vi "base color selection_N2.vi"(8 "error in":errorcluster, 11 "Sample Sequence":string="GATGATGATGATGATGAT") -> (0 "error out":errorcluster, 2 "element":string, 3 "Base All Composition":T1(array[cluster]))   [LabVIEW 2018]
panel:
  out "R STD Level array":dbl[](array[numeric])
  out "Base Species IDX array":dbl[](array[numeric])
  out "Base name array":string[](array[string])
  out "Base Color array":u32[](array[numeric])
  out "R Base Level array":dbl[](array[numeric])
  out "Base array":string[](array[string])
  out "Base_N":string
  out "Base All Composition X":T1(array[cluster])
  out "Base C":string[](array[string])
  out "Base Composition":string[](array[string])
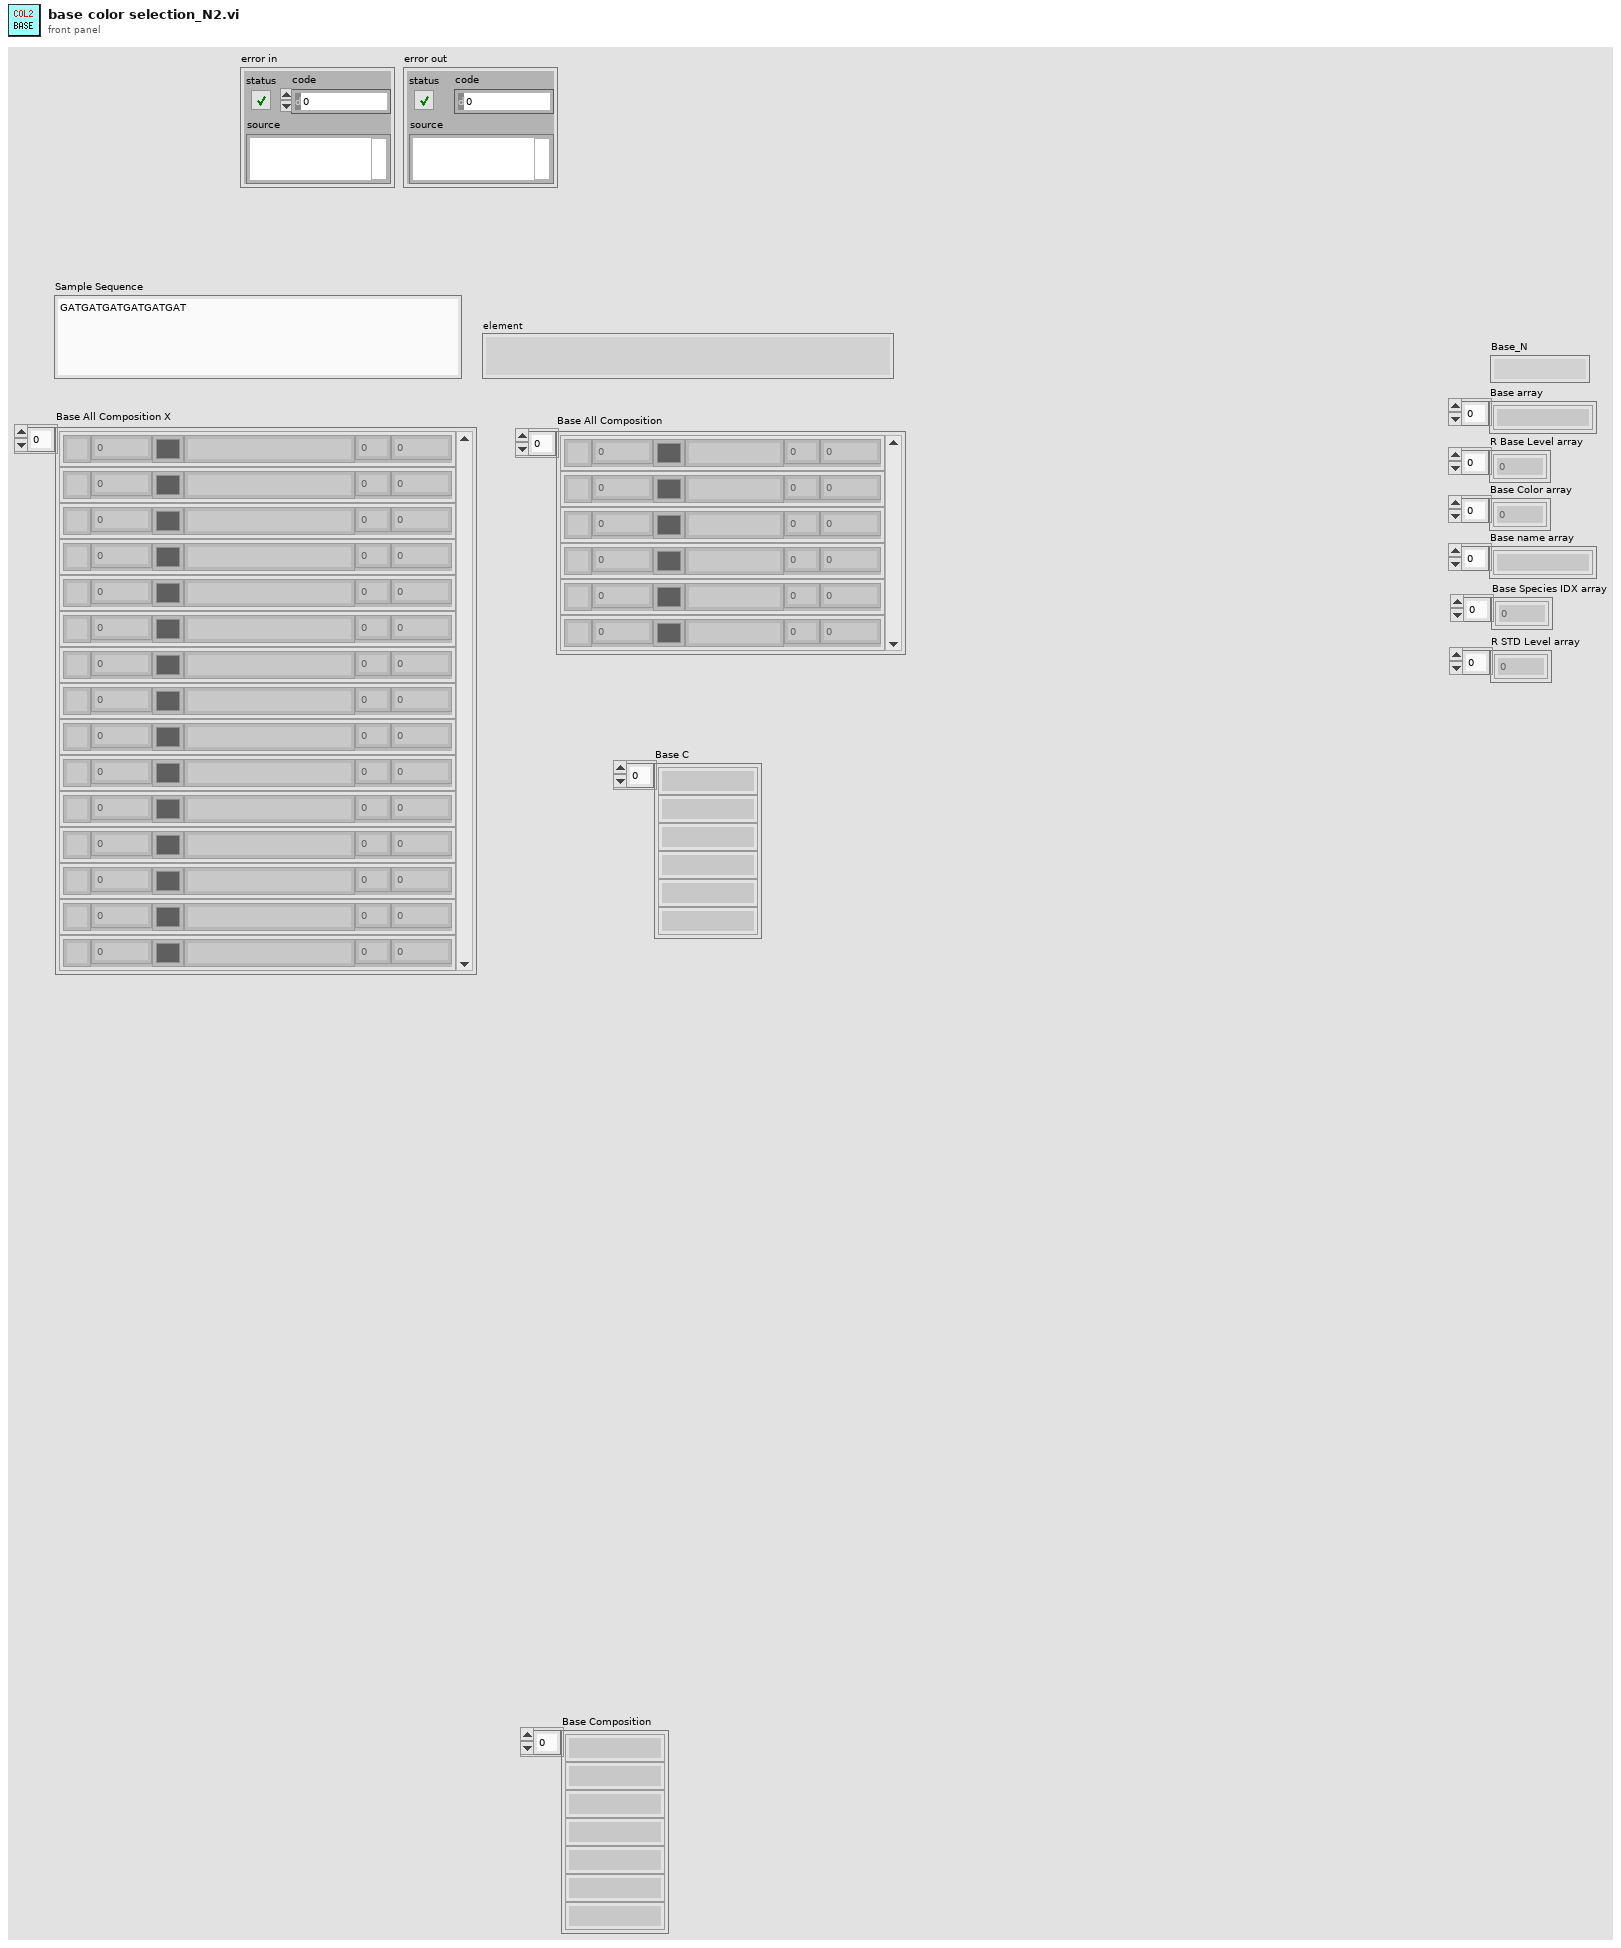
[diagram p1: front panel]
types:
  T1 = cluster{"Name":string, "Value":dbl, "Color":u32, "Name 2":string, "Value 2":dbl, "Value 3":dbl}[]
  T2 = cluster{"Name":string, "Value":dbl, "Color":u32, "Name 2":string, "Value 2":dbl, "Value 3":dbl}
  T3 = cluster{u16, "Item":cluster{"Name":string, "Value":dbl, "Color":u32, "Name 2":string, "Value 2":dbl, "Value 3":dbl}}
  T4 = cluster{u16, "Item":cluster{"Name":string, "Value":dbl, "Color":u32, "Name 2":string, "Value 2":dbl, "Value 3":dbl}}[]
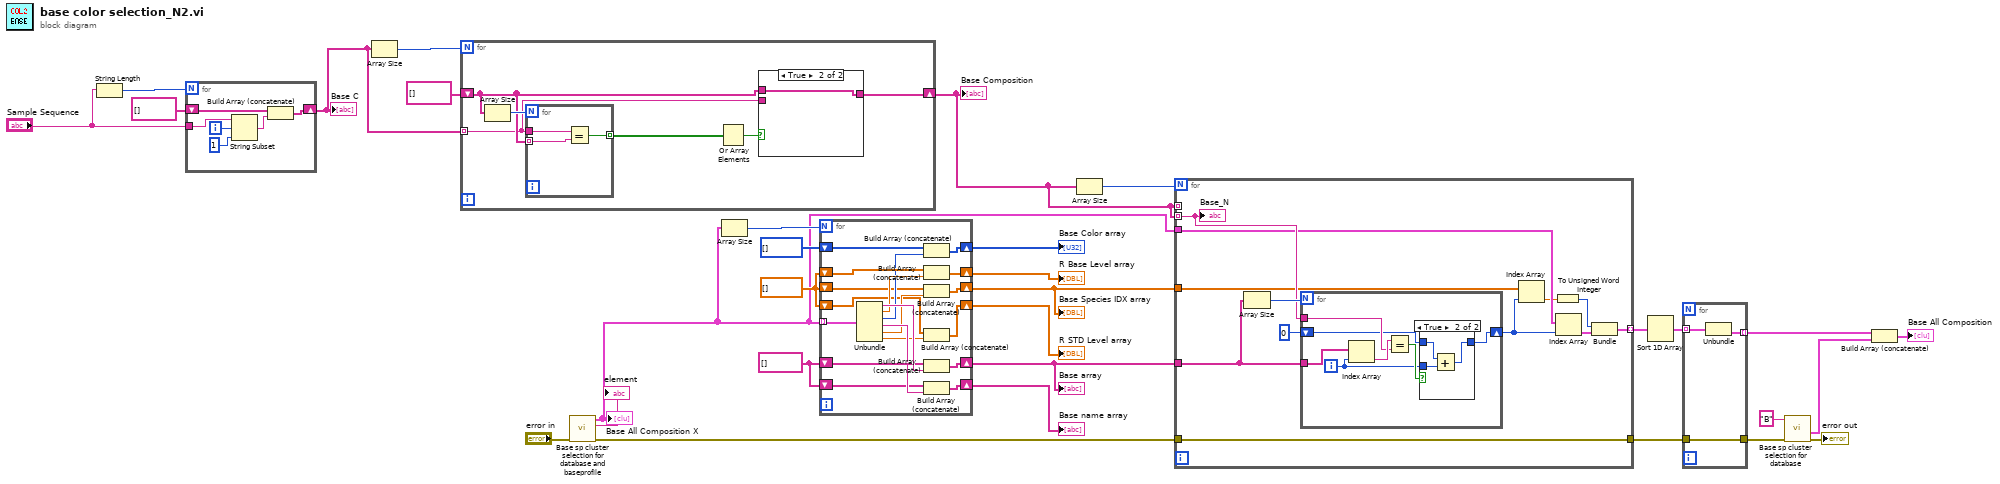
[diagram p0: block diagram]
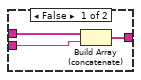
[diagram p3: hidden frame]
diagram:
  w13 = dbl[] []
  w14 = string[] []
  n1 = String Length(string="Sample Sequence") -> (length=w31:i32)
  n2 = for {
    N: w31 -> [_]
    tunnel: "Sample Sequence" -> [w35]
    shift-right: [w34] -> w26
    shift-left: string[] [] -> [w33]
    i -> [w36]
    n3 = String Subset(string=w35, offset (0)=w36, length (rest)=1 ("長さ（残り）")) -> (substring=w32:string)
    n4 = Build Array (concatenate)(w33, w32) -> (w34:string[])
  }
  "Base C" <- w26
  n5 = Array Size(array=w26) -> (size(s)=w28:i32)
  n6 = for {
    N: w28 -> [_]
    tunnel: w26 -> [w40] mode=indexing
    shift-right: [w43] -> w17
    shift-left: string[] [] -> [w41]
    n7 = Array Size(array=w41) -> (size(s)=w42:i32)
    n8 = for {
      N: w42 -> [_]
      tunnel: w41 -> [w50] mode=indexing
      tunnel: w40 -> [w49]
      tunnel: [w48] -> w39 mode=indexing
      n9 = Equal?(x=w49, y=w50) -> (x = y?=w48:bool)
    }
    n10 = Or Array Elements(Boolean array=w39) -> (logical OR=w38:bool)
    n11 = case shown="True" w38 {
      tunnel: [w46 w47] -> w43
      tunnel: w41 -> [w45 w47]
      tunnel: w40 -> [w44 _]
      frame False {
        n12 = Build Array (concatenate)(w45, w44) -> (w46:string[])
      }
      frame True {
      }
    }
  }
  "Base Composition" <- w17
  n13 = call "Base sp cluster selection for database and baseprofile.vi"("error in"="error in") -> ("error out"=w3:errorcluster, "element"=→"element":string, "Base All Composition"=w2:T1)  [unwired: 8 in]
  "Base All Composition X" <- w2
  n14 = Array Size(array=w2) -> (size(s)=w16:i32)
  n15 = for {
    N: w16 -> [_]
    tunnel: w2 -> [w69] mode=indexing
    shift-right: [w67] -> w8
    shift-left: w14 -> [w66]
    shift-right: [w65] -> w12
    shift-left: w13 -> [w63]
    shift-right: [w58] -> w11
    shift-left: u32[] [] -> [w57]
    shift-right: [w56] -> w10
    shift-left: w14 -> [w53]
    shift-right: [w55] -> w7
    shift-left: w13 -> [w54]
    shift-right: [w52] -> w9
    shift-left: w13 -> [w51]
    n16 = Unbundle(w69) -> ("Name"=w68:string, "Value"=w64:dbl, "Color"=w62:u32, "Name 2"=w61:string, "Value 2"=w60:dbl, "Value 3"=w59:dbl)
    n17 = Build Array (concatenate)(w57, w62) -> (w58:u32[])
    n18 = Build Array (concatenate)(w63, w64) -> (w65:dbl[])
    n19 = Build Array (concatenate)(w54, w60) -> (w55:dbl[])
    n20 = Build Array (concatenate)(w51, w59) -> (w52:dbl[])
    n21 = Build Array (concatenate)(w66, w68) -> (w67:string[])
    n22 = Build Array (concatenate)(w53, w61) -> (w56:string[])
  }
  "Base array" <- w8
  "R Base Level array" <- w12
  "Base Color array" <- w11
  "Base name array" <- w10
  "Base Species IDX array" <- w7
  "R STD Level array" <- w9
  n23 = Array Size(array=w17) -> (size(s)=w18:i32)
  n24 = for {
    N: w18 -> [_]
    tunnel: w17 -> [_] mode=indexing
    tunnel: w3 -> [w70]
    tunnel: [w70] -> w6
    tunnel: w8 -> [w80]
    tunnel: w17 -> [w78] mode=indexing
    tunnel: w7 -> [w77]
    tunnel: w2 -> [w76]
    tunnel: [w74] -> w5 mode=indexing
    n25 = Array Size(array=w80) -> (size(s)=w79:i32)
    n26 = for {
      N: w79 -> [_]
      tunnel: w80 -> [w83]
      tunnel: w78 -> [w87]
      shift-right: [w84] -> w72
      shift-left: 0 ("index") -> [w85]
      i -> [w82]
      n27 = Index Array(array=w83, index=w82) -> (element=w88:string)
      n28 = Equal?(x=w88, y=w87) -> (x = y?=w86:bool)
      n29 = case shown="True" w86 {
        tunnel: [w89 w91] -> w84
        tunnel: w85 -> [w89 w90]
        tunnel: w82 -> [_ w92]
        frame False {
        }
        frame True {
          n30 = Add(x=w90, y=w92) -> (x+y=w91:i32)
        }
      }
    }
    n31 = Index Array(array=w77, index=w72) -> (element=w73:dbl)
    n32 = To Unsigned Word Integer(number=w73) -> (unsigned 16bit integer=w71:u16)
    n33 = Index Array(array=w76, index=w72) -> (element=w75:T2)
    n34 = Bundle(w71, "Item"=w75) -> (w74:T3)  [unwired: 1 in]
    "Base_N" <- w78
  }
  n35 = Sort 1D Array(array=w5) -> (sorted array=w25:T4)
  n36 = for {
    tunnel: w25 -> [w95] mode=indexing
    tunnel: [w94] -> w24 mode=indexing
    tunnel: [w93] -> w20
    tunnel: w6 -> [w93]
    n37 = Unbundle(w95) -> ("Item"=w94:T2)  [unwired: 1 out]
  }
  n38 = call "Base sp cluster selection for database.vi"("error in"=w20, "Base"="B") -> ("error out"=→"error out":errorcluster, "Item"=w21:T2)  [unwired: 6 in, 2 out]
  n39 = Build Array (concatenate)(w24, w21) -> (→"Base All Composition":T1)
